vi "Create from VI.vi"(7 "Test Name":string, 8 "error in (no error)":errorcluster, 10 "Test Method VI Path":path, 11 "LUnit Test Case In":refnum<class "LUnit Test Case.lvclass">) -> (0 "error out":errorcluster, 3 "LUnit Test Case Out":refnum<class "LUnit Test Case.lvclass">)   [LabVIEW 2020, in "LUnit Test Case.lvclass"]
doc: "Create a test case object from a VI Path. Leave the test name unwired to use default."
uses:
  LUnit Test Case.lvclass
  LUnit Test Case.lvclass/LUnit Test Case.ctl
  Result/Status.ctl
  Result/Result.lvlib
  Result/Type.ctl
  Result/Result.ctl
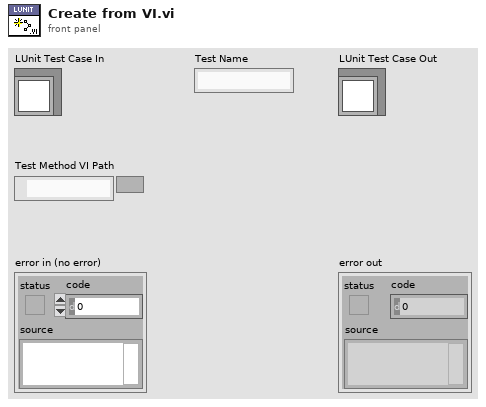
[diagram p1: front panel]
types:
  T1 = typedef "Result.lvlib/Result.ctl" = cluster{"Name":string, "Description":string, "Status":T2, "Result Type":T3, "Execution Time":dbl, "Data":cluster{"Expected":variant, "Actual":variant, "Delta":variant}}
  T2 = typedef "Result.lvlib/Status.ctl" = enum16{"", "Passed", "Failed", "Error", "Skipped", "Setup Error", "Broken", "Teardown Error"}
  T3 = typedef "Result.lvlib/Type.ctl" = enum16{"Test Case", "Test Suite", "Test Run", "Pass", "Fail", "Skip", "Pass if", "Fail if", "Pass if Error", "Fail if Error", "Pass if Equal", "Fail if Equal"}
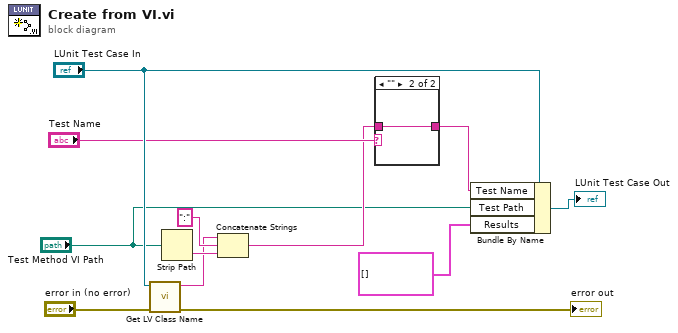
[diagram p0: block diagram]
diagram:
  n1 = call <vilib>:"Get LV Class Name.vi"("error in (no error)"="error in (no error)", "object"="LUnit Test Case In") -> ("error out"=→"error out":errorcluster, "class name"=w4:string)  [unwired: 8 in]
  n2 = Strip Path(path="Test Method VI Path") -> (name=w5:string)  [unwired: 1 out]
  n3 = Concatenate Strings(w4, ":" ("string"), w5) -> (w3:string)
  n4 = case shown="\"\"" "Test Name" {
    selector: "Test Name" -> [w13 _]
    tunnel: w3 -> [_ w14]
    tunnel: [w13 w14] -> w10
    frame Default {
    }
    frame "" {
    }
  }
  n5 = Bundle By Name(cluster="LUnit Test Case In", "Test Name"=w10, "Test Path"="Test Method VI Path", "Results"=T1[] []) -> (→"LUnit Test Case Out":refnum<class "LUnit Test Case.lvclass">)
